vi "Variant_ExtractClusterElementByName.vi"(9 "name":string, 11 "Cluster":variant) -> (1 "index":i32=-1, 2 "Element":variant, 3 "Cluster dup":variant)   [LabVIEW 2013, in "OpenVariant.lvlib"]
uses:
  OpenVariant.lvlib
  TypeDescriptor/OpenDescriptor.lvlib
  Conversions/OpenConvert.lvlib
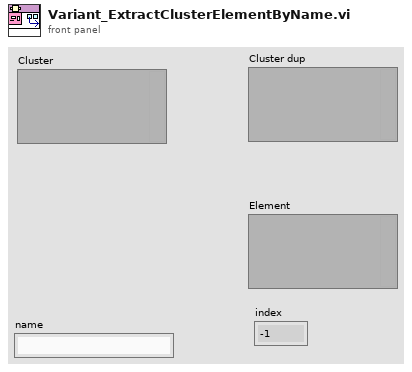
[diagram p1: front panel]
types:
  T1 = typedef "OpenDescriptor.lvlib/OpenDescriptor -- cluster.ctl" = cluster{"type descriptor":i16[], "name":string, "class":string, "data string":string}
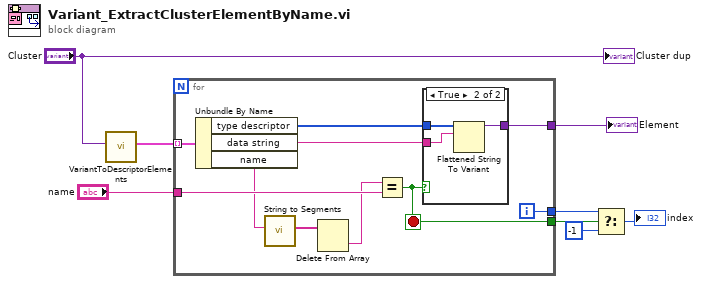
[diagram p0: block diagram]
diagram:
  n1 = call "VariantToDescriptorElements.vi"("Variant"="Cluster") -> ("Descriptors"=w1:T1[])  [unwired: 9 in, 1 out]
  n2 = for {
    tunnel: w1 -> [w18] mode=indexing
    tunnel: "name" -> [w17]
    tunnel: [w14] -> w7
    tunnel: [w13] -> w6
    tunnel: [w12] -> w5
    i -> [w12]
    stop <- w13 stop-if-true
    n3 = Unbundle By Name(w18) -> ("type descriptor"=w16:i16[], "data string"=w15:string, "name"=w10:string)
    n4 = call "String to Segments.vi"("String"=w10) -> ("Segments"=w11:string[])  [unwired: 9 in, 1 out]
    n5 = Delete From Array(array=w11) -> (deleted portion=w9:string)  [unwired: 2 in, 1 out]
    n6 = Equal?(x=w9, y=w17) -> (x = y?=w13:bool)
    n7 = case shown="True" w13 {
      tunnel: w16 -> [_ w21]
      tunnel: w15 -> [_ w20]
      tunnel: [_ w19] -> w14
      frame False {
      }
      frame True {
        n8 = Flattened String To Variant(6:w20, 7:w21) -> (3:w19:variant)  [unwired: 1 in, 1 out]
      }
    }
  }
  "Element" <- w7
  n9 = Select(t=w5, s=w6, f=-1) -> (s? t:f=→"index":i32)
  "Cluster dup" <- "Cluster"
